vi "UMLEditor RemoveStaticObjects.vi"(5 "error in (no error)":errorcluster) -> (19 "error out":errorcluster)   [LabVIEW 2020]
uses:
  <resource>/Framework/Providers/Open_GDS/UML/ClassDiagramGraph_class/ClassDiagramGraph.lvclass
  <resource>/Framework/Providers/Open_GDS/UML/SequenceDiagramGraph_class/SequenceDiagramGraph.lvclass
  <resource>/Framework/Providers/Open_GDS/UML/UseCaseDiagramGraph_class/UseCaseDiagramGraph.lvclass
  <resource>/Framework/Providers/Open_GDS/UML/StateDiagramGraph_class/StateDiagramGraph.lvclass
  <resource>/Framework/Providers/Open_GDS/UML/AbstractEdge_class/AbstractEdge.lvclass
  <resource>/Framework/Providers/Open_GDS/UML/AbstractNode_class/AbstractNode.lvclass
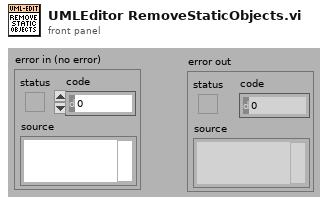
[diagram p1: front panel]
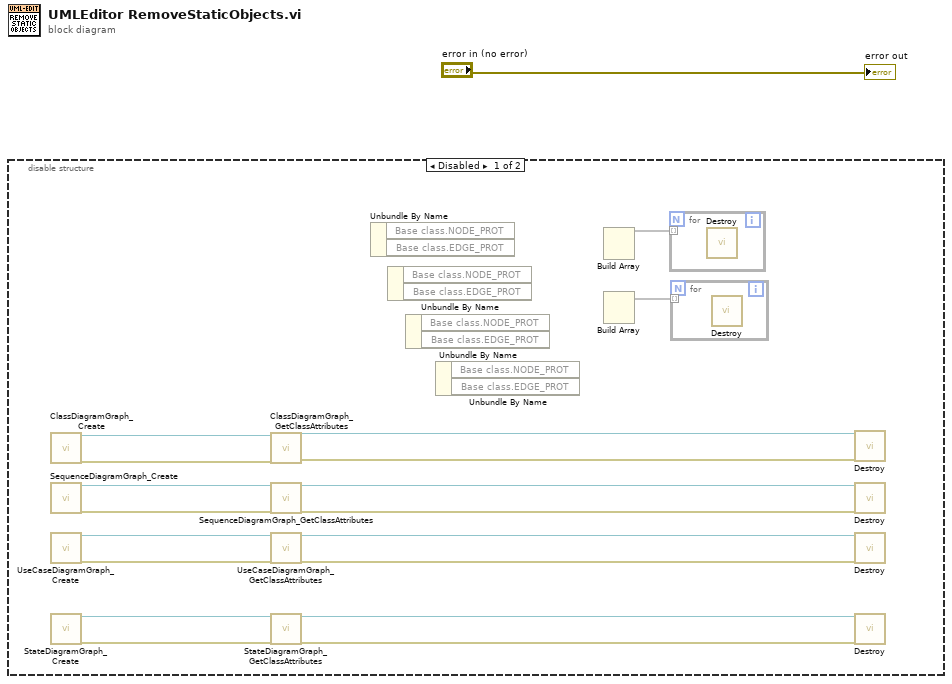
[diagram p0: block diagram]
diagram:
  n1 = disable-structure shown="Disabled" {
    frame Disabled {
      n2 = call <resource>:"ClassDiagramGraph_Create.vi"() -> ("reference out"=w19:refnum<class "ClassDiagramGraph.lvclass">, "error out"=w8:errorcluster)  [unwired: 2 in, 16 out]
      n3 = call <resource>:"SequenceDiagramGraph_Create.vi"() -> ("reference out"=w14:refnum<class "SequenceDiagramGraph.lvclass">, "error out"=w7:errorcluster)  [unwired: 2 in, 16 out]
      n4 = call <resource>:"UseCaseDiagramGraph_Create.vi"() -> ("reference out"=w13:refnum<class "UseCaseDiagramGraph.lvclass">, "error out"=w6:errorcluster)  [unwired: 2 in, 16 out]
      n5 = call <resource>:"StateDiagramGraph_Create.vi"() -> ("reference out"=w3:refnum<class "StateDiagramGraph.lvclass">, "error out"=w2:errorcluster)  [unwired: 3 in, 15 out]
      n6 = call <resource>:"ClassDiagramGraph_GetClassAttributes.vi"("reference in"=w19, "error in (no error)"=w8) -> ("reference out"=w18:refnum<class "ClassDiagramGraph.lvclass">, "error out"=w17:errorcluster)  [unwired: 16 out]
      n7 = call <resource>:"SequenceDiagramGraph_GetClassAttributes.vi"("reference in"=w14, "error in (no error)"=w7) -> ("reference out"=w12:refnum<class "SequenceDiagramGraph.lvclass">, "error out"=w11:errorcluster)  [unwired: 16 out]
      n8 = call <resource>:"UseCaseDiagramGraph_GetClassAttributes.vi"("reference in"=w13, "error in (no error)"=w6) -> ("reference out"=w10:refnum<class "UseCaseDiagramGraph.lvclass">, "error out"=w9:errorcluster)  [unwired: 16 out]
      n9 = call <resource>:"StateDiagramGraph_GetClassAttributes.vi"("reference in"=w3, "error in (no error)"=w2) -> ("reference out"=w4:refnum<class "StateDiagramGraph.lvclass">, "error out"=w5:errorcluster)  [unwired: 16 out]
      n10 = Unbundle By Name() -> ()  [unwired: 1 in, 2 out]
      n11 = Unbundle By Name() -> ()  [unwired: 1 in, 2 out]
      n12 = Unbundle By Name() -> ()  [unwired: 1 in, 2 out]
      n13 = Unbundle By Name() -> ()  [unwired: 1 in, 2 out]
      n14 = Build Array() -> (w16:void[])  [unwired: 4 in]
      n15 = Build Array() -> (w15:void[])  [unwired: 4 in]
      n16 = for {
        tunnel: w16 -> [_] mode=indexing
        n17 = call-dynamic "Destroy.vi"() -> ()  [unwired: 18 in, 2 out]
      }
      n18 = for {
        tunnel: w15 -> [_] mode=indexing
        n19 = call-dynamic "Destroy.vi"() -> ()  [unwired: 19 in, 1 out]
      }
      n20 = call-dynamic "Destroy.vi"("reference"=w18, "error in (no error)"=w17) -> ()  [unwired: 17 in, 1 out]
      n21 = call-dynamic "Destroy.vi"("reference"=w12, "error in (no error)"=w11) -> ()  [unwired: 17 in, 1 out]
      n22 = call-dynamic "Destroy.vi"("reference"=w10, "error in (no error)"=w9) -> ()  [unwired: 17 in, 1 out]
      n23 = call-dynamic "Destroy.vi"("reference"=w4, "error in (no error)"=w5) -> ()  [unwired: 17 in, 1 out]
    }
    frame Enabled {
    }
  }
  "error out" <- "error in (no error)"
